vi "DialogRenameClass.vi"(0 "ClassWriterNative.lvclass":refnum<class "ClassWriterNative.lvclass">, 1 "ClassItemRefIn":refnum<vi>, 5 "error in (no error)":errorcluster) -> (14 "ClassWriterGOOP300.lvclassOut":refnum<class "ClassWriterNative.lvclass">, 15 "ClassItemRefOut":refnum<vi>, 16 "NewClassPath":path, 17 "Cancelled":bool, 18 "RelinkWholeProject":bool, 19 "error out":errorcluster)   [LabVIEW 2020, in "ClassWriterNative.lvclass"]
uses:
  ClassWriterNative.lvclass
  5772000b-287c-4c6f-9312-1e31dd0b0ac3.vi
  <vilib>/Utility/lvfile.llb/NI_FileType.lvlib
panel:
  in  "Help":bool
  out "ProductPicture":picture
  in  "_RelinkWholeProject":bool
  in  "_ShowContextHelp":bool
  in  "_UseClassSuffix":string caption="Class Folder Suffix"
  in  "_NewClassPath":path caption="New Class Path"
  in  "_NewClassName":string caption="New Class Name"
  out "_DubName":string caption="This class already exists"
  out "_OldClassName":string caption="Old Class Name"
  in  "_Cancel":bool
  in  "_RenameClass":bool
  out "_OldClassPath":path caption="Old Class Path"
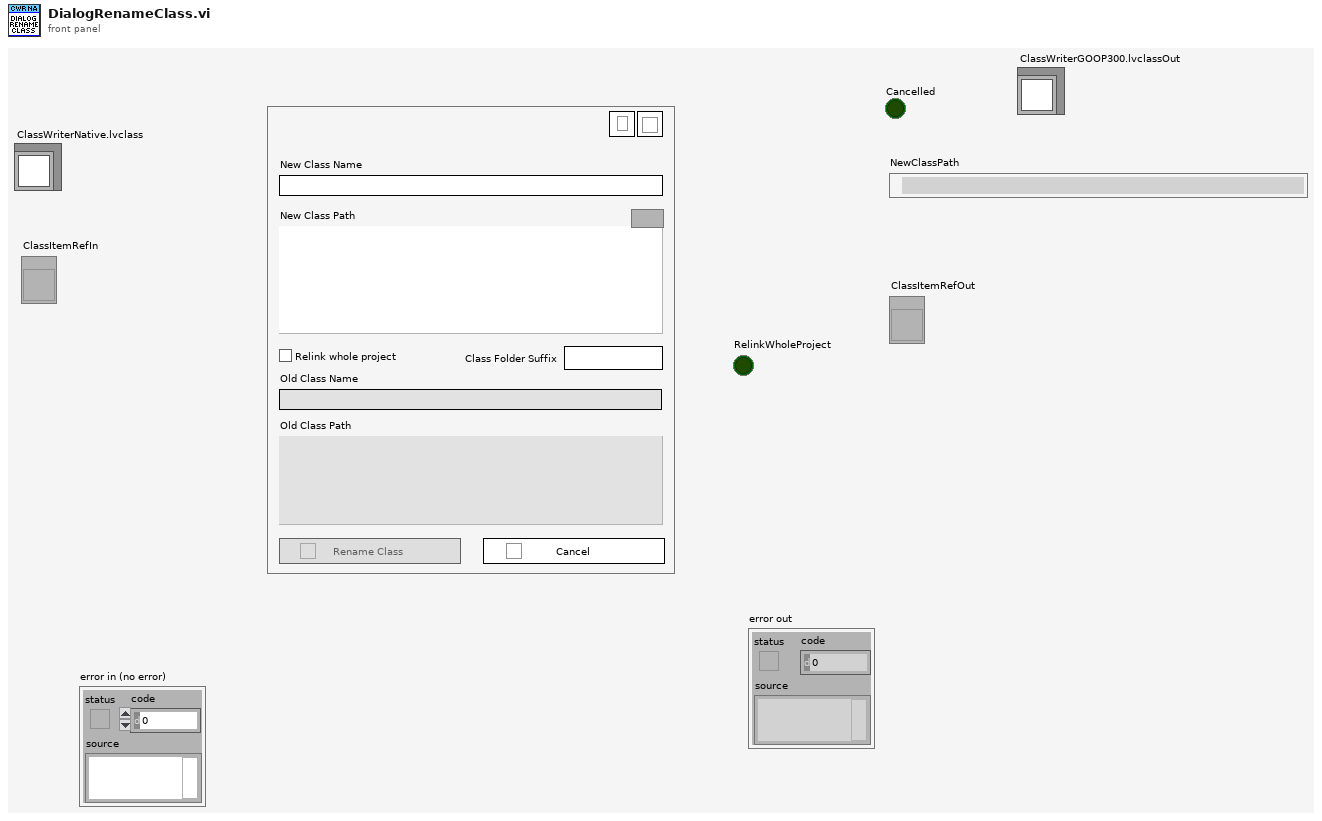
[diagram p1: front panel]
types:
  T1 = cluster{"Cancel":bool, "OrgClassPath":path, "ClassName":string, "Interface":bool}
  T2 = typedef "BaseProvider_IniFileSettings.ctl" = cluster{"ClassFolderSuffix":string, "InterfaceFolderSuffix":string, "InterfaceIcon":string, "FileNamingOption":T3, "DynamicDispatchStartValue":bool}
  T3 = typedef "BaseProvider_FileNamingOption.ctl" = enum16{"CamelCase", "Space", "Underscore"}
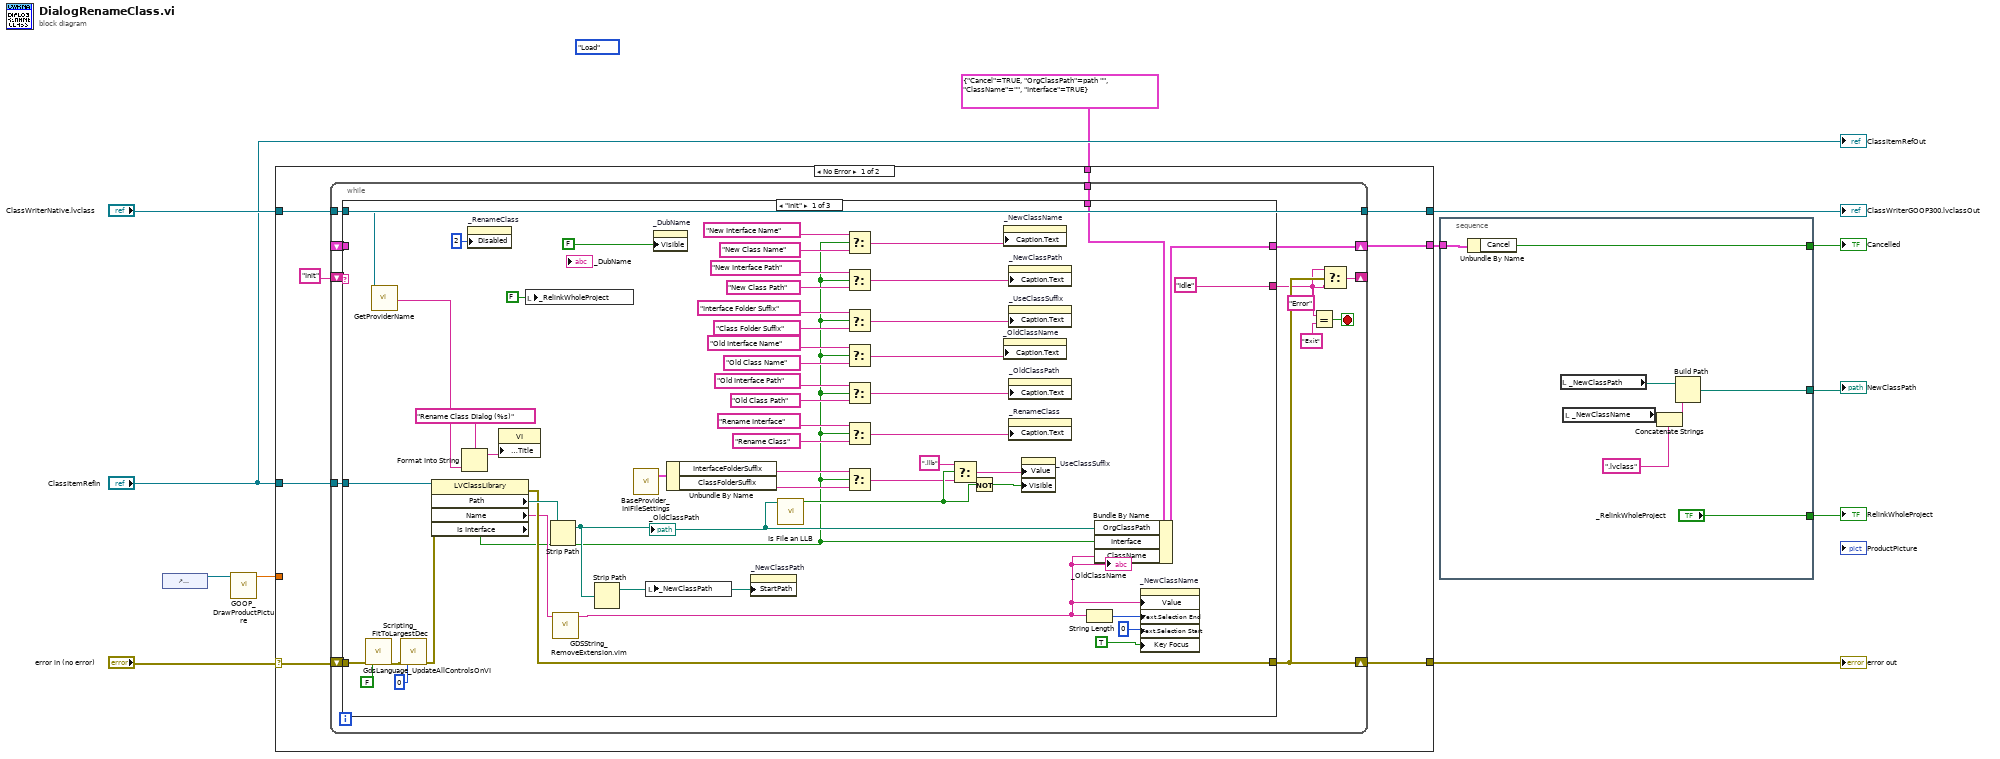
[diagram p0: block diagram]
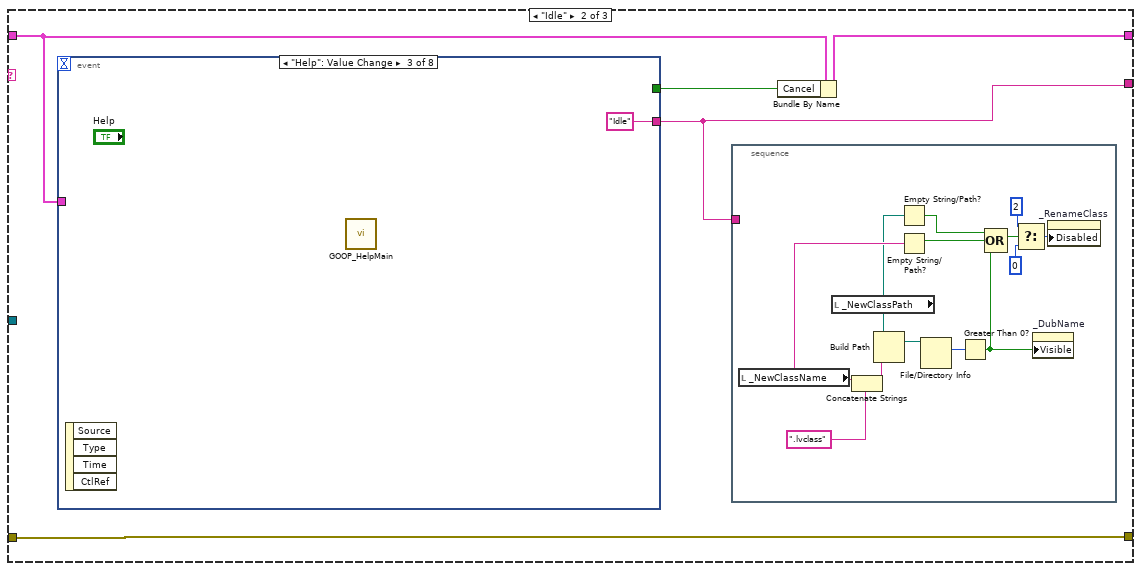
[diagram p2: hidden frame]
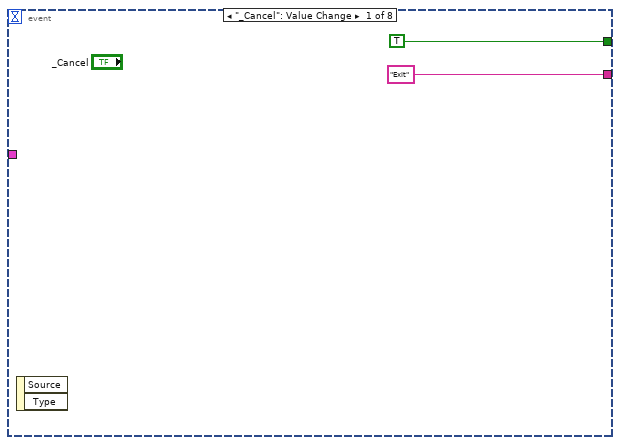
[diagram p3: hidden frame]
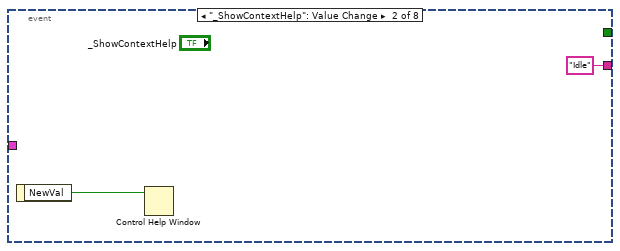
[diagram p4: hidden frame]
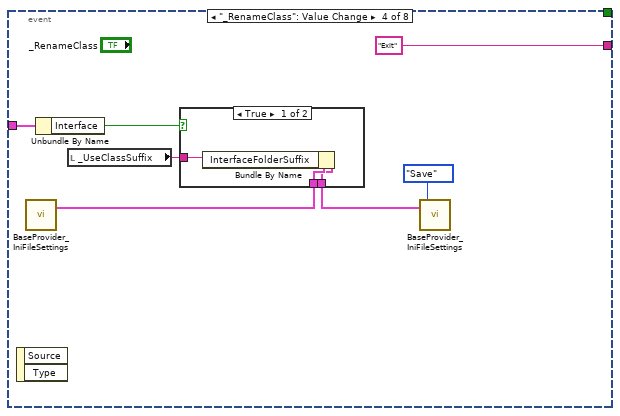
[diagram p5: hidden frame]
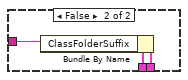
[diagram p6: hidden frame]
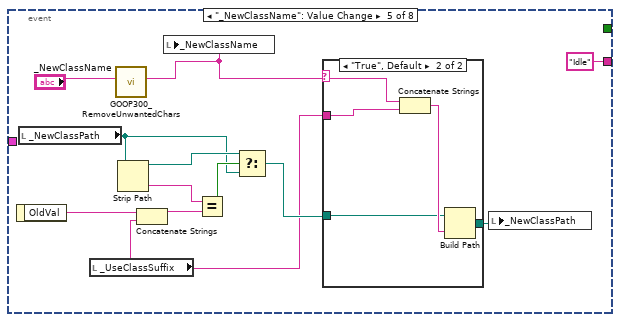
[diagram p7: hidden frame]
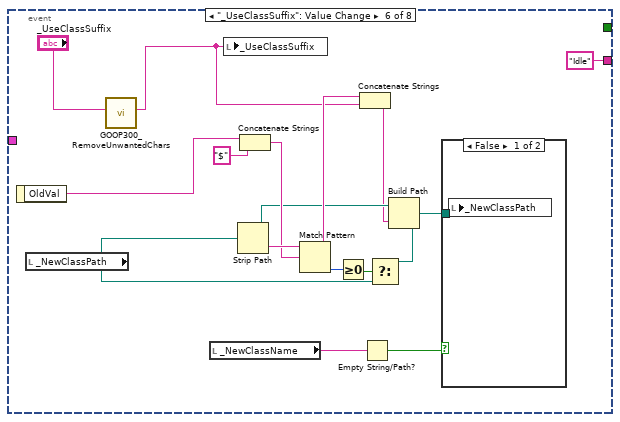
[diagram p9: hidden frame]
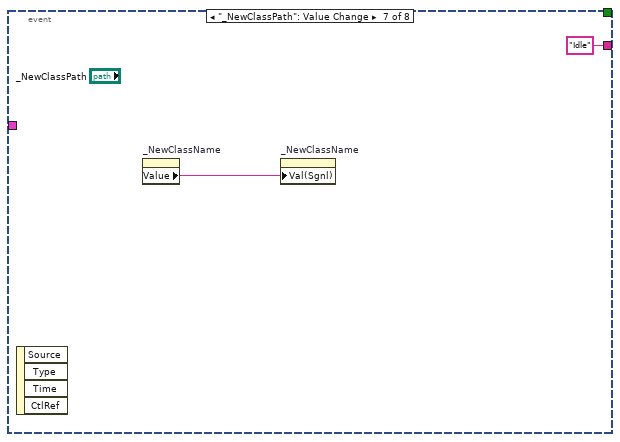
[diagram p11: hidden frame]
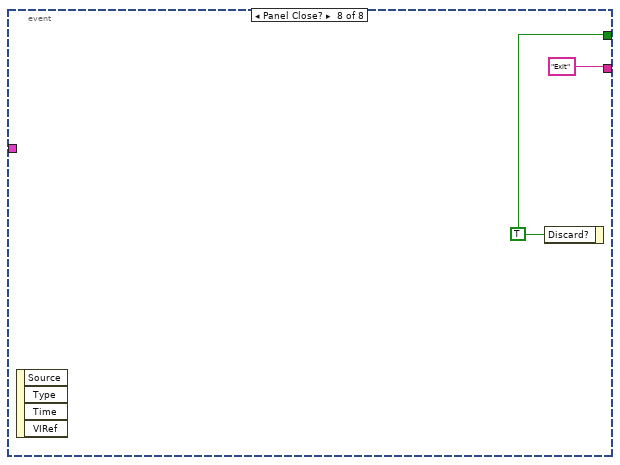
[diagram p12: hidden frame]
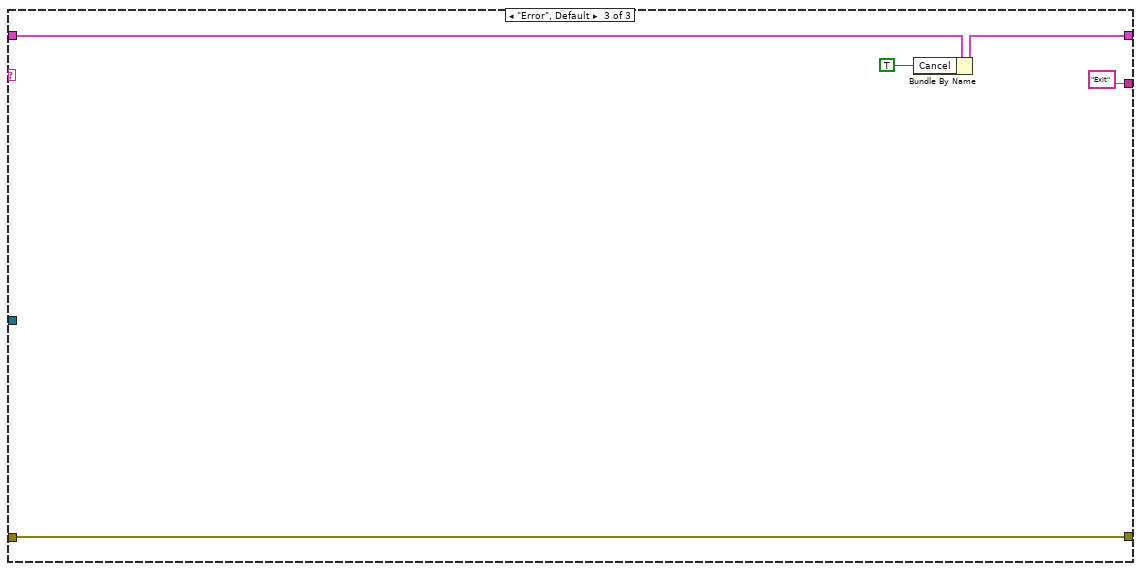
[diagram p13: hidden frame]
diagram:
  (unwired) enum16{"Read", "Load", "Save"}."Load" ("Action")
  n1 = control-ref of="ProductPicture"() -> (w2:refnum<vi>)
  n2 = call "GOOP_DrawProductPicture.vi"("ProductPictureControl"=w2) -> ("Zoom Factor"=w1:sgl)  [unwired: 10 in]
  n3 = case shown="No Error" "error in (no error)" {
    selector: "error in (no error)" -> [w20 w167]
    tunnel: "ClassWriterNative.lvclass" -> [w16 w166]
    tunnel: [w19 w167] -> w6
    tunnel: [w17 w166] -> w10
    tunnel: T1 {"Cancel"=TRUE, "OrgClassPath"=path "", "ClassName"="", "Interface"=TRUE} ("output cluster") -> [w15 _]
    tunnel: "ClassItemRefIn" -> [w14 _]
    tunnel: [w13 _] -> w9
    tunnel: w1 -> [_ _]
    frame No Error {
      n4 = while {
        shift-right: [w27] -> w19
        shift-left: w20 -> [w33]
        shift-right: [w26] -> _
        shift-left: "Init" -> [w30]
        shift-right: [w31] -> w13
        shift-left: _ -> [w32]
        tunnel: w16 -> [w23]
        tunnel: [w23] -> w17
        tunnel: w15 -> [w22]
        tunnel: w14 -> [w21]
        stop <- w28 stop-if-true
        n5 = case shown="\"Init\"" w30 {
          tunnel: w32 -> [_ w86 w163]
          tunnel: [w84 w88 w162] -> w31
          tunnel: w33 -> [w71 w90 w164]
          tunnel: [w63 w90 w164] -> w27
          tunnel: w23 -> [w72 _ _]
          tunnel: ["Idle" w89 "Exit"] -> w25
          tunnel: w22 -> [w82 _ _]
          tunnel: w21 -> [w83 _ _]
          frame "Init" {
            n6 = call "GdsLanguage_UpdateAllControlsOnVI.vi"("error in (no error)"=w71, "CreateLanguageFile(Use this to create a languageFile)"=FALSE) -> ("error out"=w62:errorcluster)  [unwired: 16 in, 1 out]
            n7 = call-dynamic "GetProviderName.vi"("ClassWriterNative in"=w72) -> ("TranslatedProviderName"=w34:string)  [unwired: 15 in, 3 out]
            n8 = call "Scripting_FitToLargestDec.vi"("error in (no error)"=w62, "border spacing (2 px)"=0) -> ("error out"=w61:errorcluster)  [unwired: 4 in, 1 out]
            n9 = property class="LVClassLibrary"(reference=w83, error in=w61) -> (error out=w63:errorcluster, "Path"=w80:path, "Name"=w59:string, "Is Interface"=w35:bool)  [unwired: 1 out]
            n10 = Format Into String(format string="Rename Class Dialog (%s)", w34) -> (resulting string=w74:string)  [unwired: 2 in, 1 out]
            n11 = property on="_RenameClass" class="Bool"("Disabled"=u8 2) -> ()  [unwired: 2 in, 2 out]
            n12 = property class="VI"("Front Panel.Title"=w74) -> ()  [unwired: 2 in, 2 out]
            n13 = local write "_RelinkWholeProject"(FALSE ("_RelinkWholeProject")) -> ()
            n14 = Strip Path(path=w80) -> (stripped path=w69:path)  [unwired: 1 out]
            "_OldClassPath" <- w69
            n15 = call "GDSString_RemoveExtension.vim"("NameWithExtension"=w59) -> ("NameWithoutExtension"=w45:string)  [unwired: 9 in, 1 out]
            "_OldClassName" <- w45
            n16 = Strip Path(path=w69) -> (stripped path=w76:path)  [unwired: 1 out]
            n17 = call "BaseProvider_IniFileSettings.vi"() -> ("IniFileSettings"=w58:T2)  [unwired: 18 in, 1 out]
            n18 = local write "_NewClassPath"(w76) -> ()
            n19 = property on="_DubName" class="Str"("Visible"=FALSE) -> ()  [unwired: 2 in, 2 out]
            n20 = Unbundle By Name(w58) -> ("InterfaceFolderSuffix"=w57:string, "ClassFolderSuffix"=w56:string)
            n21 = property on="_NewClassPath" class="Path"("StartPath"=w76) -> ()  [unwired: 2 in, 2 out]
            n22 = call <vilib>:"Is File an LLB.vi"("path"=w69) -> ("Is LLB?"=w67:bool)  [unwired: 9 in, 1 out]
            n23 = Select(t="New Interface Name" ("Caption.Text"), s=w35, f="New Class Name" ("Caption.Text")) -> (s? t:f=w55:string)
            n24 = Select(t="New Interface Path" ("Caption.Text"), s=w35, f="New Class Path" ("Caption.Text")) -> (s? t:f=w49:string)
            n25 = Select(t="Interface Folder Suffix" ("Caption.Text"), s=w35, f="Class Folder Suffix" ("Caption.Text")) -> (s? t:f=w48:string)
            n26 = Select(t="Old Interface Name" ("Caption.Text"), s=w35, f="Old Class Name" ("Caption.Text")) -> (s? t:f=w38:string)
            n27 = Select(t="Old Interface Path" ("Caption.Text"), s=w35, f="Old Class Path" ("Caption.Text")) -> (s? t:f=w42:string)
            n28 = Select(t="Rename Interface" ("Caption.Text"), s=w35, f="Rename Class" ("Caption.Text")) -> (s? t:f=w43:string)
            n29 = Select(t=w57, s=w35, f=w56) -> (s? t:f=w52:string)
            n30 = Select(t=".llb" ("y"), s=w67, f=w52) -> (s? t:f=w65:string)
            n31 = Not(x=w67) -> (.not. x?=w68:bool)
            n32 = property on="_NewClassName" class="Str"("Caption.Text"=w55) -> ()  [unwired: 2 in, 2 out]
            n33 = property on="_OldClassName" class="Str"("Caption.Text"=w38) -> ()  [unwired: 2 in, 2 out]
            n34 = property on="_NewClassPath" class="Path"("Caption.Text"=w49) -> ()  [unwired: 2 in, 2 out]
            n35 = property on="_UseClassSuffix" class="Str"("Caption.Text"=w48) -> ()  [unwired: 2 in, 2 out]
            n36 = property on="_OldClassPath" class="Path"("Caption.Text"=w42) -> ()  [unwired: 2 in, 2 out]
            n37 = property on="_RenameClass" class="Bool"("Caption.Text"=w43) -> ()  [unwired: 2 in, 2 out]
            n38 = property on="_UseClassSuffix" class="Str"("Value"=w65, "Visible"=w68) -> ()  [unwired: 2 in, 2 out]
            n39 = String Length(string=w45) -> (length=w75:i32)
            n40 = Bundle By Name(cluster=w82, "OrgClassPath"=w69, "Interface"=w35, "ClassName"=w45) -> (w84:T1)
            n41 = property on="_NewClassName" class="Str"("Value"=w45, "Text.Selection End"=w75, "Text.Selection Start"=u32 0 ("Text.Selection:Start"), "Key Focus"=TRUE) -> ()  [unwired: 2 in, 2 out]
          }
          frame "Idle" {
            n42 = event shown="[2] \"Help\": Value Change" {
              selector: _ -> [_ _ _ _ _ _ _ _]
              dyn-events: _ -> [_ _ _ _ _ _ _ _]
              timeout: _ -> [_ _ _ _ _ _ _ _]
              tunnel: ["Exit" "Idle" "Idle" "Exit" "Idle" "Idle" "Idle" "Exit"] -> w89
              tunnel: [TRUE _ _ _ _ _ _ w160] -> w87
              tunnel: w86 -> [_ _ _ w110 _ _ _ _]
              event "_Cancel": Value Change {
                n43 = event-data() -> ()  [unwired: 1 in, 2 out]
              }
              event "_ShowContextHelp": Value Change {
                n44 = event-data() -> ("NewVal"=w106:bool)  [unwired: 1 in]
                n45 = Control Help Window(1:w106) -> ()  [unwired: 1 in]
              }
              event "Help": Value Change {
                n46 = event-data() -> ()  [unwired: 1 in, 4 out]
                n47 = call "GOOP_HelpMain.vi"() -> ()  [unwired: 12 in]
              }
              event "_RenameClass": Value Change {
                n48 = event-data() -> ()  [unwired: 1 in, 2 out]
                n49 = call "BaseProvider_IniFileSettings.vi"() -> ("IniFileSettings"=w113:T2)  [unwired: 18 in, 1 out]
                n50 = Unbundle By Name(w110) -> ("Interface"=w109:bool)
                n51 = local read "_UseClassSuffix"() -> (w111:string)
                n52 = case shown="True" w109 {
                  tunnel: w113 -> [w118 w121]
                  tunnel: [w117 w120] -> w112
                  tunnel: w111 -> [w116 w119]
                  frame True {
                    n53 = Bundle By Name(cluster=w118, "InterfaceFolderSuffix"=w116) -> (w117:T2)
                  }
                  frame False {
                    n54 = Bundle By Name(cluster=w121, "ClassFolderSuffix"=w119) -> (w120:T2)
                  }
                }
                n55 = call "BaseProvider_IniFileSettings.vi"("IniFileSettings"=w112, "Action"=enum16{"Read", "Load", "Save"}."Save") -> ()  [unwired: 16 in, 2 out]
              }
              event "_NewClassName": Value Change {
                n56 = event-data() -> ("OldVal"=w125:string)  [unwired: 1 in]
                n57 = local read "_NewClassPath"() -> (w122:path)
                n58 = local read "_UseClassSuffix"() -> (w124:string)
                n59 = call "GOOP300_RemoveUnwantedChars.vi"("StringIn"="_NewClassName") -> ("StringOut"=w126:string)  [unwired: 10 in]
                n60 = Strip Path(path=w122) -> (stripped path=w129:path, name=w131:string)
                n61 = Concatenate Strings(w125, w124) -> (w132:string)
                n62 = local write "_NewClassName"(w126) -> ()
                n63 = Equal?(x=w131, y=w132) -> (x = y?=w130:bool)
                n64 = Select(t=w129, s=w130, f=w122) -> (s? t:f=w128:path)
                n65 = case shown="\"True\", Default" w126 {
                  selector: w126 -> [_ w135]
                  tunnel: [w134 w139] -> w123
                  tunnel: w124 -> [_ w138]
                  tunnel: w128 -> [w134 w136]
                  frame "" {
                  }
                  frame "True", Default {
                    n66 = Concatenate Strings(w135, w138) -> (w137:string)
                    n67 = Build Path(base path=w136, name or relative path=w137) -> (appended path=w139:path)
                  }
                }
                n68 = local write "_NewClassPath"(w123) -> ()
              }
              event "_UseClassSuffix": Value Change {
                n69 = event-data() -> ("OldVal"=w142:string)  [unwired: 1 in]
                n70 = local read "_NewClassPath"() -> (w145:path)
                n71 = call "GOOP300_RemoveUnwantedChars.vi"("StringIn"="_UseClassSuffix") -> ("StringOut"=w146:string)  [unwired: 10 in]
                n72 = local read "_NewClassName"() -> (w141:string)
                n73 = local write "_UseClassSuffix"(w146) -> ()
                n74 = Strip Path(path=w145) -> (stripped path=w148:path, name=w154:string)
                n75 = Concatenate Strings(w142, "$" ("string")) -> (w152:string)
                n76 = Match Pattern(string=w154, regular expression=w152) -> (before substring=w149:string, offset past match=w153:i32)  [unwired: 1 in, 2 out]
                n77 = Greater Or Equal To 0?(x=w153) -> (x >= 0?=w150:bool)
                n78 = Concatenate Strings(w149, w146) -> (w147:string)
                n79 = Empty String/Path?(string/path=w141) -> (empty?=w140:bool)
                n80 = Build Path(base path=w148, name or relative path=w147) -> (appended path=w144:path)
                n81 = Select(t=w144, s=w150, f=w145) -> ()  [unwired: 1 out]
                n82 = case shown="False" w140 {
                  tunnel: w144 -> [w156 _]
                  frame False {
                    n83 = local write "_NewClassPath"(w156) -> ()
                  }
                  frame True {
                  }
                }
              }
              event "_NewClassPath": Value Change {
                n84 = event-data() -> ()  [unwired: 1 in, 4 out]
                n85 = property on="_NewClassName" class="Str"() -> ("Value"=w157:string)  [unwired: 2 in, 2 out]
                n86 = property on="_NewClassName" class="Str"("Val(Sgnl)"=w157) -> ()  [unwired: 2 in, 2 out]
              }
              event Panel Close? {
                w160 = TRUE ("Discard?")
                n87 = event-data() -> ()  [unwired: 1 in, 4 out]
                n88 = event-data("Discard?"=w160) -> ()  [unwired: 1 in, 1 out]
              }
            }
            n89 = stacked-sequence {
              tunnel: w89 -> [_]
              frame #0 {
                n90 = local read "_NewClassName"() -> (w94:string)
                n91 = local read "_NewClassPath"() -> (w92:path)
                n92 = Concatenate Strings(w94, ".lvclass" ("string")) -> (w98:string)
                n93 = Build Path(base path=w92, name or relative path=w98) -> (appended path=w97:path)
                n94 = Empty String/Path?(string/path=w92) -> (empty?=w91:bool)
                n95 = Empty String/Path?(string/path=w94) -> (empty?=w93:bool)
                n96 = File/Directory Info(path=w97) -> (size=w96:i64)  [unwired: 1 in, 6 out]
                n97 = Greater Than 0?(x=w96) -> (x > 0?=w95:bool)
                n98 = Compound Arithmetic op=OR(w91, w93, w95) -> (w100:bool)
                n99 = Select(t=u8 2, s=w100, f=u8 0 ("Disabled")) -> (s? t:f=w103:u8)
                n100 = property on="_DubName" class="Str"("Visible"=w95) -> ()  [unwired: 2 in, 2 out]
                n101 = property on="_RenameClass" class="Bool"("Disabled"=w103) -> ()  [unwired: 2 in, 2 out]
              }
            }
            n102 = Bundle By Name(cluster=w86, "Cancel"=w87) -> (w88:T1)
          }
          frame "Error", Default {
            n103 = Bundle By Name(cluster=w163, "Cancel"=TRUE) -> (w162:T1)
          }
        }
        n104 = Equal?(x=w25, y="Exit") -> (x = y?=w28:bool)
        n105 = Select(t="Error", s=w27, f=w25) -> (s? t:f=w26:string)
      }
    }
    frame Error {
    }
  }
  "ClassWriterGOOP300.lvclassOut" <- w10
  "error out" <- w6
  n106 = stacked-sequence {
    tunnel: w9 -> [w174]
    tunnel: [w175] -> w8
    tunnel: [w169] -> w4
    tunnel: ["_RelinkWholeProject"] -> w3
    frame #0 {
      n107 = Unbundle By Name(w174) -> ("Cancel"=w175:bool)
      n108 = local read "_NewClassPath"() -> (w173:path)
      n109 = local read "_NewClassName"() -> (w172:string)
      n110 = Concatenate Strings(w172, ".lvclass" ("string")) -> (w171:string)
      n111 = Build Path(base path=w173, name or relative path=w171) -> (appended path=w169:path)
    }
  }
  "Cancelled" <- w8
  "NewClassPath" <- w4
  "RelinkWholeProject" <- w3
  "ClassItemRefOut" <- "ClassItemRefIn"
